vi "Write a Json.vi"() -> ()   [LabVIEW 2021]
uses:
  json class.lvclass
panel:
  out "Pretty JSON String":string="{\r  \"System\": {\r    \"active\": true,\r    \"installationDate\": \"2026-11-04T17:10:22.000Z\",\r    \"location\": {\r      \"coordinates\": {\r        \"latitude\": 10,\r        \"longitude\": -66.9036\r      },\r      \"plant\": \"North\"\r    },\r    \"name\": \"Test_Station_01\",\r    \"version\": \"2.4.1\"\r  },\r  \"hardware\": {\r    \"controller\": {\r      \"ip\": \"192.168.1.50\",\r      \"model\": \"cRIO-9045\",\r      \"operatingSystem\": \"NI Linux Real-Time\"\r    },\r    \"modules\": {\r      \"MyArray\": [\r        {\r          \"channels\": {\r            \"id\": \"ai0\",\r            \"name\": \"Inlet_Pressure\"\r          },\r          \"model\": \"NI-9205\",\r          \"slot\": 0,\r          \"type\": \"AI\"\r        },\r        {\r          \"channels\": {\r            \"id\": \"ai0\",\r            \"name\": \"Inlet_Pressure\"\r          },\r          \"model\": \"NI-9401\",\r          \"slot\": 1,\r          \"type\": \"DIO\"\r        }\r      ]\r    }\r  }\r}"
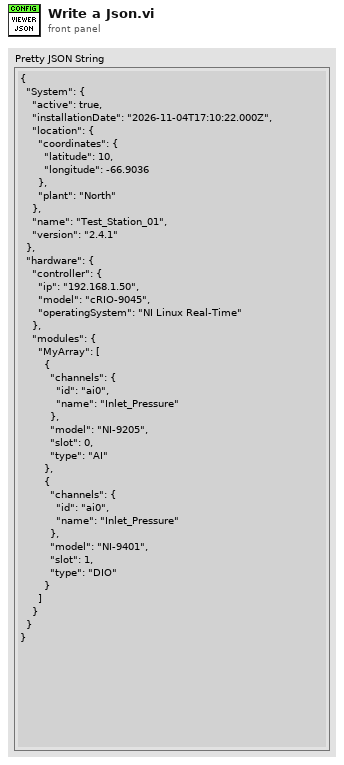
[diagram p1: front panel]
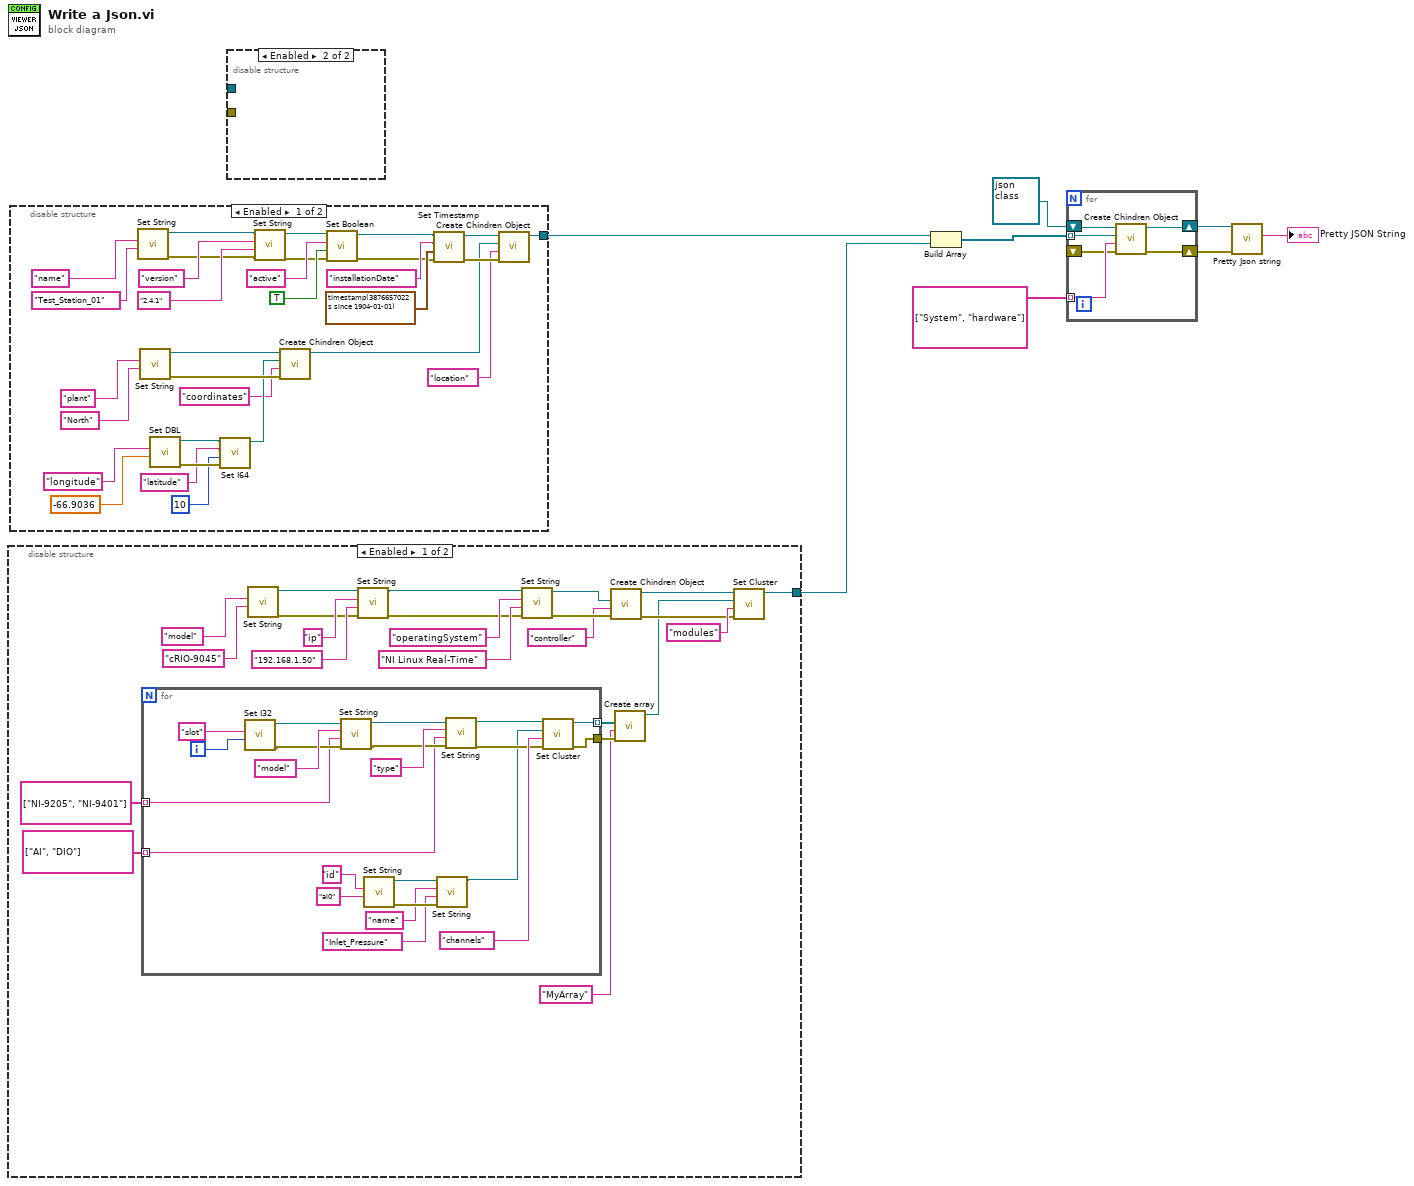
[diagram p0: block diagram]
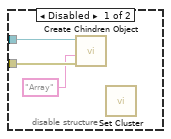
[diagram p4: hidden frame]
diagram:
  n1 = disable-structure shown="Enabled" {
    disable-tunnel: [w17 _] -> w1
    frame Enabled {
      n2 = for {
        tunnel: [w44] -> w13 mode=indexing
        tunnel: string[] ["NI-9205", "NI-9401"] ("Name") -> [w40] mode=indexing
        tunnel: string[] ["AI", "DIO"] ("Name") -> [w39] mode=indexing
        tunnel: [w32] -> w10
        i -> [w45]
        n3 = call "Set I32.vi"("Value"=w45, "Name"="slot") -> ("error out"=w46:errorcluster, "json class out"=w47:refnum<class "json class.lvclass">)  [unwired: 8 in]
        n4 = call "Set String.vi"("error in (no error)"=w46, "String"=w40, "Name"="model", "json class in"=w47) -> ("error out"=w50:errorcluster, "json class out"=w51:refnum<class "json class.lvclass">)  [unwired: 6 in]
        n5 = call "Set String.vi"("String"="ai0" ("Name"), "Name"="id") -> ("error out"=w36:errorcluster, "json class out"=w37:refnum<class "json class.lvclass">)  [unwired: 8 in]
        n6 = call "Set String.vi"("error in (no error)"=w36, "String"="Inlet_Pressure" ("Name"), "Name"="name", "json class in"=w37) -> ("json class out"=w33:refnum<class "json class.lvclass">)  [unwired: 6 in, 1 out]
        n7 = call "Set String.vi"("error in (no error)"=w50, "String"=w39, "Name"="type", "json class in"=w51) -> ("error out"=w42:errorcluster, "json class out"=w49:refnum<class "json class.lvclass">)  [unwired: 6 in]
        n8 = call "Set Cluster.vi"("error in (no error)"=w42, "Name"="channels", "Cluster Class"=w33, "json class in"=w49) -> ("error out"=w32:errorcluster, "json class out"=w44:refnum<class "json class.lvclass">)  [unwired: 6 in]
      }
      n9 = call "Set String.vi"("String"="cRIO-9045" ("Name"), "Name"="model") -> ("error out"=w26:errorcluster, "json class out"=w27:refnum<class "json class.lvclass">)  [unwired: 8 in]
      n10 = call "Set String.vi"("error in (no error)"=w26, "String"="192.168.1.50" ("Name"), "Name"="ip", "json class in"=w27) -> ("error out"=w23:errorcluster, "json class out"=w22:refnum<class "json class.lvclass">)  [unwired: 6 in]
      n11 = call "Set String.vi"("error in (no error)"=w23, "String"="NI Linux Real-Time" ("Name"), "Name"="operatingSystem", "json class in"=w22) -> ("error out"=w21:errorcluster, "json class out"=w19:refnum<class "json class.lvclass">)  [unwired: 6 in]
      n12 = call "Create Chindren Object.vi"("error in (no error)"=w21, "Name"="controller", "Children Object"=w19) -> ("error out"=w15:errorcluster, "json class out"=w18:refnum<class "json class.lvclass">)  [unwired: 7 in]
      n13 = call "Create array.vi"("error in (no error)"=w10, "Name"="MyArray", "ArrayObject"=w13) -> ("json class out"=w14:refnum<class "json class.lvclass">)  [unwired: 7 in, 1 out]
      n14 = call "Set Cluster.vi"("error in (no error)"=w15, "Name"="modules", "Cluster Class"=w14, "json class in"=w18) -> ("json class out"=w17:refnum<class "json class.lvclass">)  [unwired: 6 in, 1 out]
    }
    frame Disabled {
    }
  }
  n15 = disable-structure shown="Enabled" {
    disable-tunnel: [w54 _] -> w7
    frame Enabled {
      n16 = call "Set String.vi"("String"="Test_Station_01" ("Name"), "Name"="name") -> ("error out"=w73:errorcluster, "json class out"=w74:refnum<class "json class.lvclass">)  [unwired: 8 in]
      n17 = call "Set String.vi"("String"="North" ("Name"), "Name"="plant") -> ("error out"=w58:errorcluster, "json class out"=w59:refnum<class "json class.lvclass">)  [unwired: 8 in]
      n18 = call "Set DBL.vi"("Value"=-66.9036, "Name"="longitude") -> ("error out"=w84:errorcluster, "json class out"=w82:refnum<class "json class.lvclass">)  [unwired: 8 in]
      n19 = call "Set I64.vi"("error in (no error)"=w84, "Value"=i64 10, "Name"="latitude", "json class in"=w82) -> ("json class out"=w57:refnum<class "json class.lvclass">)  [unwired: 6 in, 1 out]
      n20 = call "Set String.vi"("error in (no error)"=w73, "String"="2.4.1" ("Name"), "Name"="version", "json class in"=w74) -> ("error out"=w70:errorcluster, "json class out"=w69:refnum<class "json class.lvclass">)  [unwired: 6 in]
      n21 = call "Create Chindren Object.vi"("error in (no error)"=w58, "Name"="coordinates", "Children Object"=w57, "json class in"=w59) -> ("json class out"=w55:refnum<class "json class.lvclass">)  [unwired: 6 in, 1 out]
      n22 = call "Set Boolean.vi"("error in (no error)"=w70, "Boolean"=TRUE, "Name"="active", "json class in"=w69) -> ("error out"=w65:errorcluster, "json class out"=w66:refnum<class "json class.lvclass">)  [unwired: 6 in]
      n23 = call "Set Timestamp.vi"("error in (no error)"=w65, "Time Stamp"=timestamp(3876657022 s since 1904-01-01), "Name"="installationDate", "json class in"=w66) -> ("error out"=w64:errorcluster, "json class out"=w63:refnum<class "json class.lvclass">)  [unwired: 6 in]
      n24 = call "Create Chindren Object.vi"("error in (no error)"=w64, "Name"="location", "Children Object"=w55, "json class in"=w63) -> ("json class out"=w54:refnum<class "json class.lvclass">)  [unwired: 6 in, 1 out]
    }
    frame Disabled {
    }
  }
  n25 = disable-structure shown="Enabled" {
    disable-tunnel: _ -> [w87 _]
    disable-tunnel: _ -> [w86 _]
    frame Disabled {
      n26 = call "Create Chindren Object.vi"("error in (no error)"=w86, "Name"="Array", "json class in"=w87) -> ()  [unwired: 7 in, 2 out]
      n27 = call "Set Cluster.vi"() -> ()  [unwired: 10 in, 2 out]
    }
    frame Enabled {
    }
  }
  n28 = Build Array(w7, w1) -> (w2:refnum<class "json class.lvclass">[])
  n29 = for {
    shift-right: [w92] -> w4
    shift-left: refnum<class "json class.lvclass"> refnum ("json class out") -> [w93]
    tunnel: string[] ["System", "hardware"] ("Name") -> [w91] mode=indexing
    shift-right: [w90] -> w3
    shift-left: _ -> [w89]
    tunnel: w2 -> [w88] mode=indexing
    n30 = call "Create Chindren Object.vi"("error in (no error)"=w89, "Name"=w91, "Children Object"=w88, "json class in"=w93) -> ("error out"=w90:errorcluster, "json class out"=w92:refnum<class "json class.lvclass">)  [unwired: 6 in]
  }
  n31 = call "Pretty Json string.vi"("error in (no error)"=w3, "json class in"=w4) -> ("Pretty JSON String"=→"Pretty JSON String":string)  [unwired: 8 in, 1 out]
